vi "Insert Panel at Index.vi"(7 "Close Removed (T)":bool=TRUE, 8 "error in (no error)":errorcluster, 9 "2D Index":T1, 10 "ArrayPanel":refnum<class "ArrayPanel.lvclass">, 11 "2DArrayManager in":refnum<class "2DArrayManager.lvclass">) -> (0 "error out":errorcluster, 1 "Element Replaced":bool, 2 "Replaced Element":refnum<class "ArrayPanel.lvclass">, 3 "2DArrayManager out":refnum<class "2DArrayManager.lvclass">)   [LabVIEW 2020, in "OOPanel.lvlib" / "2DArrayManager.lvclass"]
uses:
  2DArrayManager.lvclass
  ArrayPanel/ArrayPanel.lvclass
  2D Index.ctl
  2DArrayManager.lvclass/2DArrayManager.ctl
  ArrayPanel/ArrayPanel.lvclass/ArrayPanel.ctl
  2DPanelBlank/2DPanelBlank.lvclass
  ec524e60-b0c9-4dc9-b7a4-63c787fc97ef.vi
  <vilib>/Comparison/Equal/Equal Functor/Equal Functor.lvclass
  OOPanel.lvlib
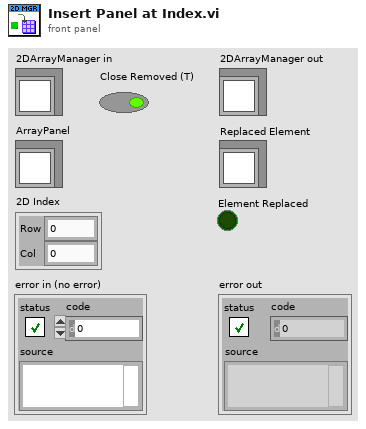
[diagram p1: front panel]
types:
  T1 = typedef "OOPanel.lvlib/2D Index.ctl" = cluster{"Row":i32, "Col":i32}
  T2 = typedef "OOPanel.lvlib/2DArrayManager.lvclass/State.ctl" = cluster{"Scroll":T3, "Scroll Max":T3, "Top-Left Index":T1, "H Scroll Sync":refnum<user-event>, "V Scroll Sync":refnum<user-event>, "Sync":bool, "H Scroll Vis":bool, "V Scroll Vis":bool, "Blank Pool":refnum<queue>}
  T3 = typedef "OOPanel.lvlib/2D Position.ctl" = cluster{"H":i32, "V":i32}
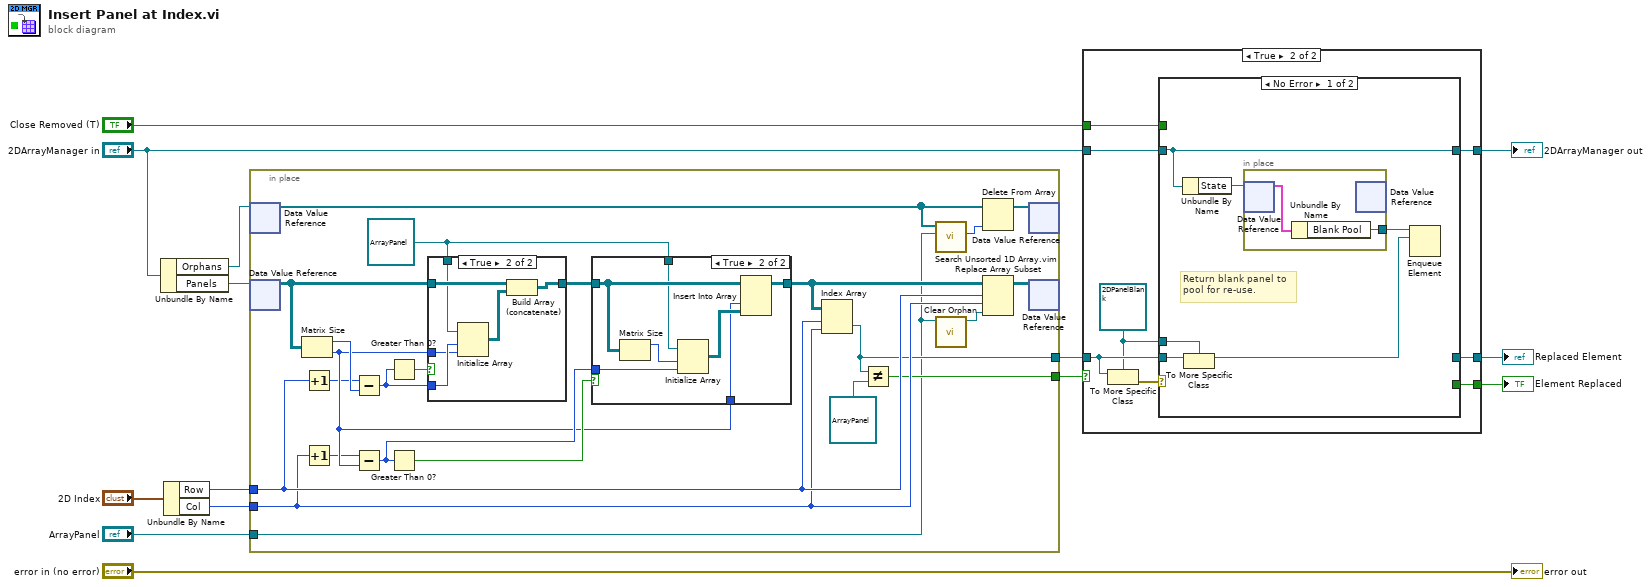
[diagram p0: block diagram]
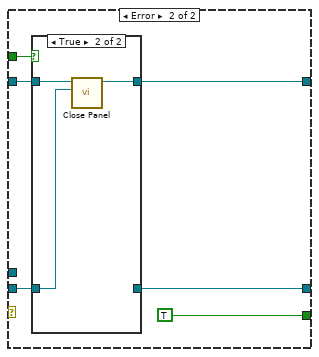
[diagram p5: hidden frame]
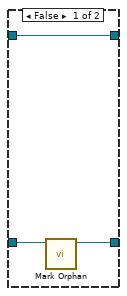
[diagram p6: hidden frame]
diagram:
  n1 = Unbundle By Name("2DArrayManager in") -> ("Orphans"=w5:refnum<data-value>, "Panels"=w12:refnum<data-value>)
  n2 = Unbundle By Name("2D Index") -> ("Row"=w11:i32, "Col"=w10:i32)
  n3 = in-place {
    in-place-border: w11 -> [w27]
    in-place-border: w10 -> [w26]
    in-place-border: "ArrayPanel" -> [w21]
    in-place-border: [w24] -> w8
    in-place-border: [w23] -> w7
    w15 = refnum<class "ArrayPanel.lvclass"> refnum ("OOPanel.lvlib:ArrayPanel.lvclass")
    n4 = in-place-dvr #1(w5) -> (w20:refnum<class "ArrayPanel.lvclass">[])  [unwired: 1 out]
    n5 = in-place-dvr #2(w12) -> (w34:refnum<class "ArrayPanel.lvclass">[][])  [unwired: 1 out]
    n6 = Matrix Size(0:w34) -> (1:w37:i32, 2:w29:i32)
    n7 = Increment(x=w27) -> (x+1=w17:i32)
    n8 = Increment(x=w26) -> (x+1=w16:i32)
    n9 = Subtract(x=w17, y=w37) -> (x-y=w35:i32)
    n10 = Subtract(x=w16, y=w29) -> (x-y=w30:i32)
    n11 = Greater Than 0?(x=w35) -> (x > 0?=w36:bool)
    n12 = Greater Than 0?(x=w30) -> (x > 0?=w31:bool)
    n13 = case shown="True" w36 {
      tunnel: w35 -> [_ w44]
      tunnel: w34 -> [w38 w42]
      tunnel: w29 -> [_ w43]
      tunnel: [w38 w40] -> w33
      tunnel: w15 -> [_ w39]
      frame False {
      }
      frame True {
        n14 = Initialize Array(w39, w44, w43) -> (w41:refnum<class "ArrayPanel.lvclass">[][])
        n15 = Build Array (concatenate)(w42, w41) -> (w40:refnum<class "ArrayPanel.lvclass">[][])
      }
    }
    n16 = case shown="True" w31 {
      tunnel: w33 -> [w45 w50]
      tunnel: [w45 w48] -> w28
      tunnel: w30 -> [_ w51]
      tunnel: w29 -> [_ w47]
      tunnel: w15 -> [_ w46]
      frame False {
      }
      frame True {
        n17 = Matrix Size(0:w50) -> (1:w52:i32)  [unwired: 1 out]
        n18 = Initialize Array(w46, w52, w51) -> (w49:refnum<class "ArrayPanel.lvclass">[][])
        n19 = Insert Into Array(array=w50, index (col)=w47, new element=w49) -> (w48:refnum<class "ArrayPanel.lvclass">[][])  [unwired: 1 in]
      }
    }
    n20 = Index Array(array=w28, index (row)=w27, index (col)=w26) -> (element=w23:refnum<class "ArrayPanel.lvclass">)
    n21 = Not Equal?(x=w23, y=refnum<class "ArrayPanel.lvclass"> refnum ("OOPanel.lvlib:ArrayPanel.lvclass")) -> (x != y?=w24:bool)
    n22 = call "Search Unsorted 1D Array.vim"("element"=w21, "unsorted 1D array"=w20) -> ("index of element"=w19:i32)  [unwired: 9 in]
    n23 = call "Clear Orphan.vi"("ArrayPanel in"=w21) -> ("ArrayPanel out"=w22:refnum<class "ArrayPanel.lvclass">)  [unwired: 9 in, 1 out]
    n24 = Delete From Array(array=w20, index=w19) -> (array with subset deleted=w18:refnum<class "ArrayPanel.lvclass">[])  [unwired: 1 in, 1 out]
    n25 = Replace Array Subset(array=w28, new element=w22, index (row)=w27, index (col)=w26) -> (w32:refnum<class "ArrayPanel.lvclass">[][])
    n26 = in-place-dvr #1(w18) -> ()  [unwired: 2 out]
    n27 = in-place-dvr #2(w32) -> ()  [unwired: 2 out]
  }
  n28 = case shown="True" w8 {
    tunnel: w7 -> [_ w56]
    tunnel: [_ w61] -> w6
    tunnel: "Close Removed (T)" -> [_ w60]
    tunnel: "2DArrayManager in" -> [w53 w59]
    tunnel: [w53 w58] -> w2
    tunnel: [_ w54] -> w1
    frame False {
    }
    frame True {
      w55 = refnum<class "2DPanelBlank.lvclass"> refnum ("OOPanel.lvlib:2DPanelBlank.lvclass")
      n29 = To More Specific Class(target class=w55, reference=w56) -> (error out=w57:errorcluster)  [unwired: 1 in, 1 out]
      n30 = case shown="No Error" w57 {
        tunnel: [_ w75] -> w61
        tunnel: w60 -> [_ w74]
        tunnel: w59 -> [w62 w73]
        tunnel: [w62 w72] -> w58
        tunnel: w56 -> [w67 w71]
        tunnel: w55 -> [w66 _]
        tunnel: [_ TRUE] -> w54
        frame No Error {
          # "Return blank panel to pool for re-use."
          n31 = Unbundle By Name(w62) -> ("State"=w65:refnum<data-value>)
          n32 = To More Specific Class(target class=w66, reference=w67) -> (specific class reference=w64:refnum<class "2DPanelBlank.lvclass">)  [unwired: 1 in, 1 out]
          n33 = in-place {
            in-place-border: [w68] -> w63
            n34 = in-place-dvr #3(w65) -> (w69:T2)  [unwired: 1 out]
            n35 = Unbundle By Name(w69) -> ("Blank Pool"=w68:refnum<queue>)
            n36 = in-place-dvr #3() -> ()  [unwired: 1 in, 2 out]
          }
          n37 = Enqueue Element(queue=w63, element=w64) -> ()  [unwired: 2 in, 3 out]
        }
        frame Error {
          n38 = case shown="True" w74 {
            tunnel: w71 -> [w78 w81]
            tunnel: [w77 _] -> w75
            tunnel: w73 -> [w76 w80]
            tunnel: [w76 w79] -> w72
            frame False {
              n39 = call "Mark Orphan.vi"("ArrayPanel in"=w78) -> ("ArrayPanel out"=w77:refnum<class "ArrayPanel.lvclass">)  [unwired: 9 in, 1 out]
            }
            frame True {
              n40 = call "Close Panel.vi"("ArrayPanel"=w81, "2DArrayManager in"=w80) -> ("2DArrayManager out"=w79:refnum<class "2DArrayManager.lvclass">)  [unwired: 8 in, 1 out]
            }
          }
        }
      }
    }
  }
  "2DArrayManager out" <- w2
  "Element Replaced" <- w1
  "Replaced Element" <- w6
  "error out" <- "error in (no error)"
